vi "TI_Proyecto3_avance_sinMyDAQ.vi"() -> ()   [LabVIEW 2025]
uses:
  <vilib>/Analysis/NI_AALBase.lvlib
panel:
  out "Salida DAC":dbl
  out "Valor entrada DAC":u32
  out "Entrada DAC":bool[](array[boolean])
  out "Salida SPI":i16[](array[numeric])
  out "Entrada SPI":i16[](array[numeric])
  out "reversed array":bool[](array[boolean])
  out "Valor binario":dbl
  out "Valor de la muestra":dbl
  out "Muestra actual":dbl
  out "Muestras":i32
  out "Señal senoidal":dbl[](array[numeric])
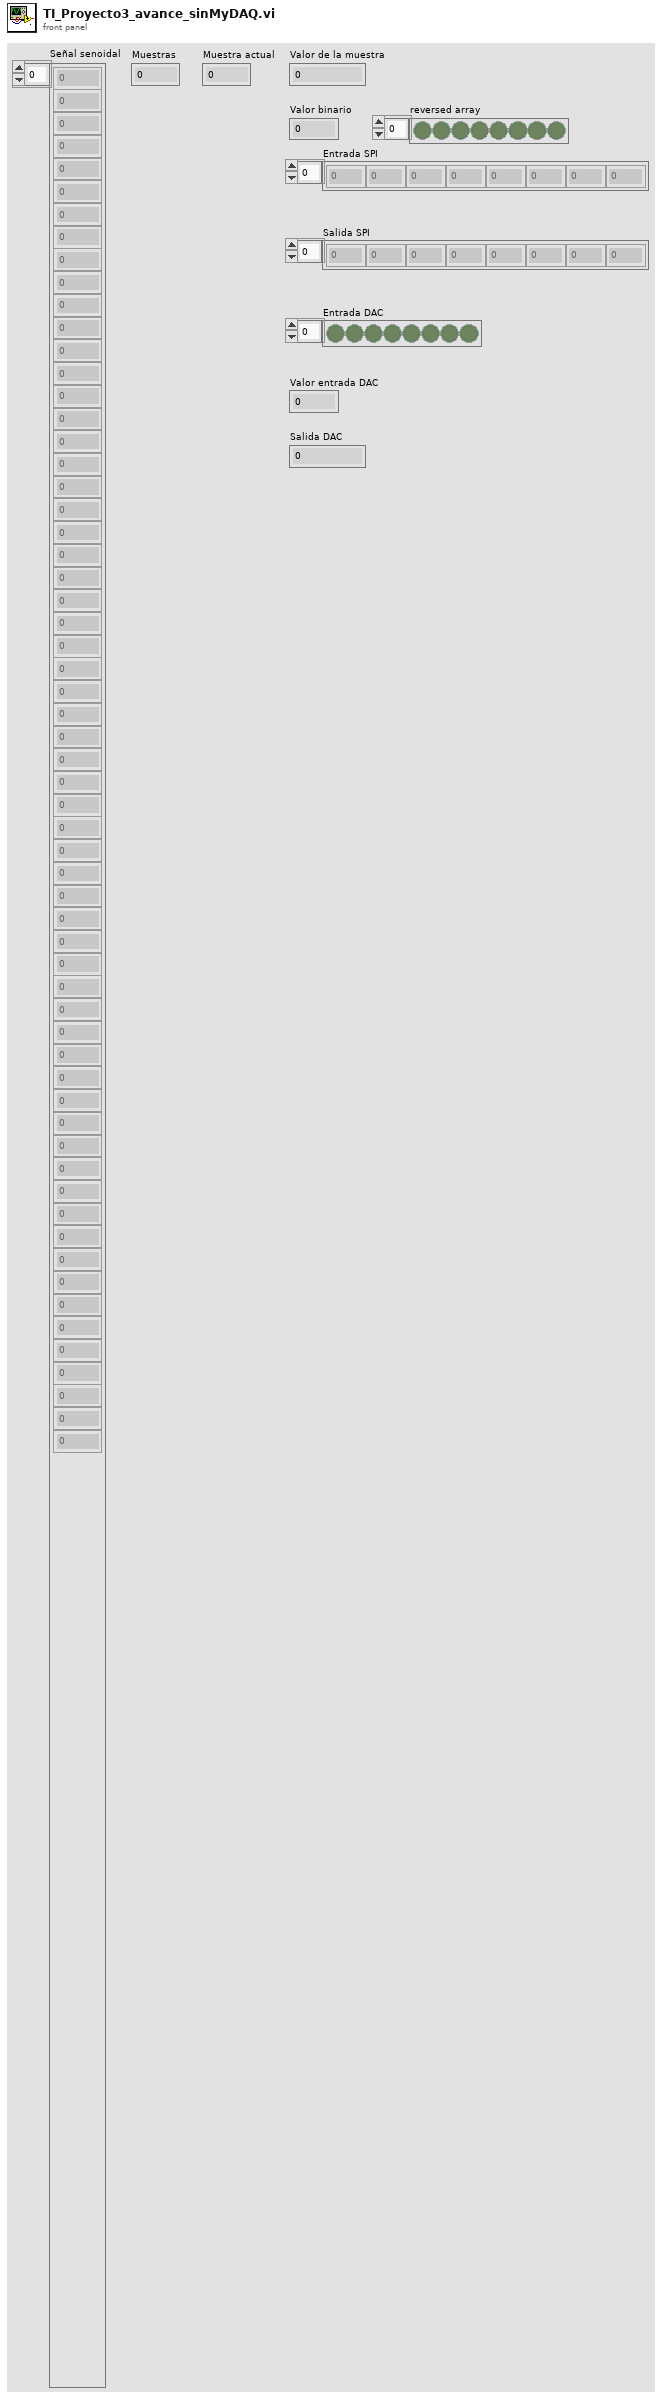
[diagram p1: front panel]
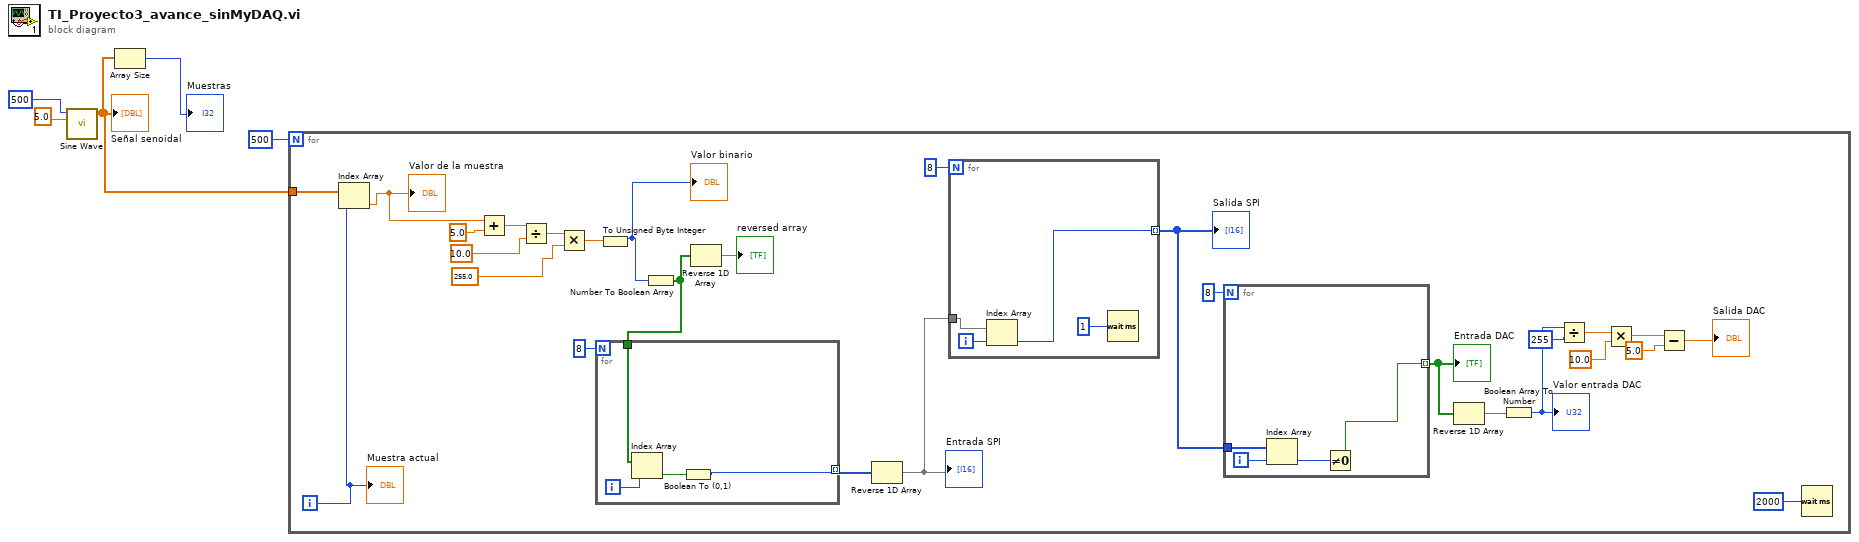
[diagram p0: block diagram]
diagram:
  n1 = call <vilib>:"Sine Wave.vi"("samples"=500, "amplitude"=5.0) -> ("sine wave"=w3:dbl[])  [unwired: 3 in, 2 out]
  "Señal senoidal" <- w3
  n2 = Array Size(array=w3) -> (size(s)=→"Muestras":i32)
  n3 = for {
    N: 500 -> [_]
    tunnel: w3 -> [w33]
    i -> [w32]
    n4 = Index Array(array=w33, index=w32) -> (element=w30:dbl)
    "Valor de la muestra" <- w30
    n5 = Add(x=w30, y=5.0) -> (x+y=w28:dbl)
    n6 = Divide(x=w28, y=10.0) -> (x/y=w26:dbl)
    n7 = Multiply(x=w26, y=255.0) -> (x*y=w24:dbl)
    n8 = To Unsigned Byte Integer(number=w24) -> (unsigned 8bit integer=w23:u8)
    "Valor binario" <- w23
    n9 = Number To Boolean Array(number=w23) -> (Boolean array=w20:bool[])
    n10 = for {
      N: 8 -> [_]
      tunnel: w20 -> [w45]
      tunnel: [w42] -> w19 mode=indexing
      i -> [w43]
      n11 = Index Array(array=w45, index=w43) -> (element=w44:bool)
      n12 = Boolean To (0,1)(Boolean=w44) -> (0, 1=w42:i16)
    }
    n13 = Reverse 1D Array(array=w20) -> (reversed array=→"reversed array":bool[])
    n14 = Reverse 1D Array(array=w19) -> (reversed array=w17:i16[])
    "Entrada SPI" <- w17
    n15 = for {
      N: 8 -> [_]
      tunnel: w17 -> [w40]
      tunnel: [w38] -> w15 mode=indexing
      i -> [w41]
      n16 = Index Array(array=w40, index=w41) -> (element=w38:i16)
      n17 = Wait (ms)(milliseconds to wait=u32 1) -> ()  [unwired: 1 out]
    }
    "Salida SPI" <- w15
    n18 = for {
      N: 8 -> [_]
      tunnel: w15 -> [w36]
      tunnel: [w34] -> w13 mode=indexing
      i -> [w37]
      n19 = Index Array(array=w36, index=w37) -> (element=w35:i16)
      n20 = Not Equal To 0?(x=w35) -> (x != 0?=w34:bool)
    }
    "Entrada DAC" <- w13
    n21 = Reverse 1D Array(array=w13) -> (reversed array=w14:bool[])
    n22 = Boolean Array To Number(Boolean array=w14) -> (number=w7:u32)
    "Valor entrada DAC" <- w7
    n23 = Divide(x=w7, y=u32 255) -> (x/y=w12:dbl)
    n24 = Multiply(x=w12, y=10.0) -> (x*y=w10:dbl)
    n25 = Subtract(x=w10, y=5.0) -> (x-y=→"Salida DAC":dbl)
    n26 = Wait (ms)(milliseconds to wait=u32 2000) -> ()  [unwired: 1 out]
    "Muestra actual" <- w32
  }
